vi "Init Events.vi"(8 "error in (no error)":errorcluster, 11 "Engine in":refnum<class "Engine.lvclass">) -> (0 "error out":errorcluster, 3 "Engine out":refnum<class "Engine.lvclass">)   [LabVIEW 2020, in "TSnax.lvlib" / "Engine.lvclass"]
uses:
  Engine.lvclass
  Open SequenceFile Request.ctl
  File Load Options.ctl
  SequenceFile/SequenceFile.lvclass
  SequenceFile Response.ctl
  VariableContainer Request.ctl
  VariableContainer Type.ctl
  PropertyObject/PropertyObject.lvclass
  VariableContainer Response.ctl
  New Execution Request.ctl
  Execution Options.ctl
  Execution Response.ctl
  Execution/Execution.lvclass
  Execution Report Request.ctl
  Report Response.ctl
  Report/Report.lvclass
  New SequenceFile Request.ctl
  Engine.lvclass/Engine.ctl
  TSnax.lvlib
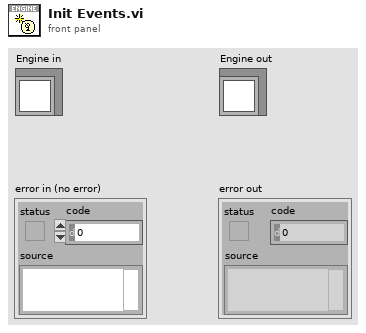
[diagram p1: front panel]
types:
  T1 = typedef "TSnax.lvlib/Engine.lvclass/New SequenceFile Request.ctl" = cluster{"Notifier":refnum<notifier>}
  T2 = typedef "TSnax.lvlib/Engine.lvclass/Execution Report Request.ctl" = cluster{"Execution":refnum<class "Execution.lvclass">, "Notifier":refnum<notifier>}
  T3 = typedef "TSnax.lvlib/Engine.lvclass/New Execution Request.ctl" = cluster{"Options":T4, "Notifier":refnum<notifier>}
  T4 = typedef "TSnax.lvlib/Execution Options.ctl" = cluster{"Use Default Model (T)":bool, "Release Related References (T)":bool}
  T5 = typedef "TSnax.lvlib/Engine.lvclass/VariableContainer Request.ctl" = cluster{"Type":T6, "Scope":refnum<class "PropertyObject.lvclass">, "Lookup String":string, "Notifier":refnum<notifier>}
  T6 = typedef "TSnax.lvlib/Engine.lvclass/VariableContainer Type.ctl" = enum16{"StationGlobals", "TemporaryGlobals", "NewPropertyObject", "SubProperty"}
  T7 = typedef "TSnax.lvlib/Engine.lvclass/Open SequenceFile Request.ctl" = cluster{"File Path":path, "File Load Options":T8, "Current SeqFile":refnum<class "SequenceFile.lvclass">, "Notifier":refnum<notifier>}
  T8 = typedef "TSnax.lvlib/File Load Options.ctl" = cluster{"Use Search Dirs? (T)":bool, "Conflict as Error? (T)":bool, "Check Station Model? (F)":bool, "Preload Modules? (T)":bool, "Skip Load Callback? (F)":bool, "Reload if Loaded? (F)":bool}
  T9 = typedef "TSnax.lvlib/Engine.lvclass/Incoming Events.ctl" = cluster{"Stop Daemon":refnum<user-event>, "Debug Line":refnum<user-event>, "Open SequenceFile":refnum<user-event>, "PropertyObject":refnum<user-event>, "New Execution":refnum<user-event>, "Execution Report":refnum<user-event>, "New SequenceFile":refnum<user-event>}
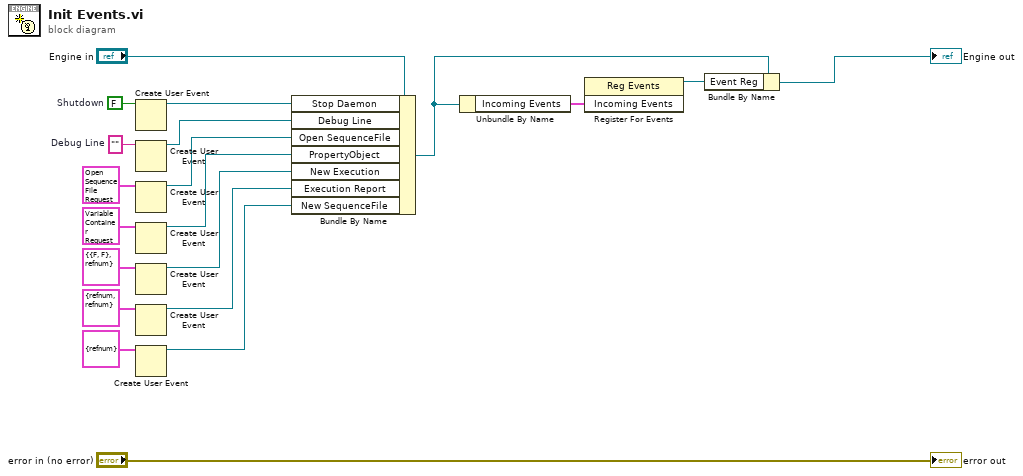
[diagram p0: block diagram]
diagram:
  w12 = ""  # Debug Line
  w18 = FALSE  # Shutdown
  n1 = Create User Event(user event datatype=w18) -> (user event=w17:refnum<user-event>)  [unwired: 1 in, 1 out]
  n2 = Create User Event(user event datatype=w12) -> (user event=w11:refnum<user-event>)  [unwired: 1 in, 1 out]
  n3 = Create User Event(user event datatype=T7 {"File Path"=path "", "File Load Options"={"Use Search Dirs? (T)"=TRUE, "Conflict as Error? (T)"=TRUE, "Check Station Model? (F)"=FALSE, "Preload Modules? (T)"=TRUE, "Skip Load Callback? (F)"=FALSE, "Reload if Loaded? (F)"=FALSE}, "Current SeqFile"=refnum, "Notifier"=refnum} ("Open SequenceFile Request")) -> (user event=w9:refnum<user-event>)  [unwired: 1 in, 1 out]
  n4 = Create User Event(user event datatype=T5 {"Type"=enum."StationGlobals", "Scope"=refnum, "Lookup String"="", "Notifier"=refnum} ("VariableContainer Request")) -> (user event=w7:refnum<user-event>)  [unwired: 1 in, 1 out]
  n5 = Create User Event(user event datatype=T3 {"Options"={"Use Default Model (T)"=FALSE, "Release Related References (T)"=FALSE}, "Notifier"=refnum} ("New Execution Request")) -> (user event=w5:refnum<user-event>)  [unwired: 1 in, 1 out]
  n6 = Create User Event(user event datatype=T2 {"Execution"=refnum, "Notifier"=refnum} ("Execution Report Request")) -> (user event=w3:refnum<user-event>)  [unwired: 1 in, 1 out]
  n7 = Create User Event(user event datatype=T1 {"Notifier"=refnum} ("New SequenceFile Request")) -> (user event=w1:refnum<user-event>)  [unwired: 1 in, 1 out]
  n8 = Bundle By Name(cluster="Engine in", "Stop Daemon"=w17, "Debug Line"=w11, "Open SequenceFile"=w9, "PropertyObject"=w7, "New Execution"=w5, "Execution Report"=w3, "New SequenceFile"=w1) -> (w16:refnum<class "Engine.lvclass">)
  n9 = Unbundle By Name(w16) -> ("Incoming Events"=w15:T9)
  n10 = register-events(w15) -> (reference out=w13:refnum<event-registration>)  [unwired: 2 in, 1 out]
  n11 = Bundle By Name(cluster=w16, "Event Reg"=w13) -> (→"Engine out":refnum<class "Engine.lvclass">)
  "error out" <- "error in (no error)"
